vi "Read Value Defaults.vi"(11 "Effect Interface in":refnum<class "Effect Interface.lvclass">) -> (1 "Value2":T1, 2 "Value1":T1, 3 "Effect Interface out":refnum<class "Effect Interface.lvclass">)   [LabVIEW 2019, in "Effect Interface.lvlib" / "Effect Interface.lvclass"]
uses:
  Effect Interface.lvclass
  Effect Interface.lvclass/Effect Interface.ctl
  Packed Libraries/Audio Processing.lvlibp/Value Properties.ctl
  Packed Libraries/Audio Processing.lvlibp
  Packed Libraries/Audio Processing.lvlibp/Value Cluster.ctl
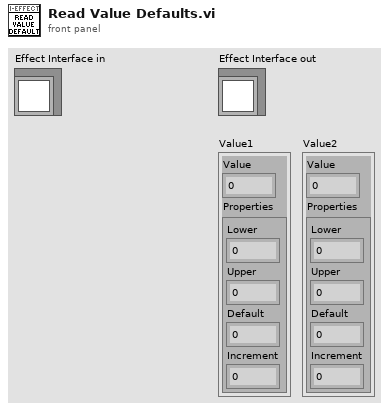
[diagram p1: front panel]
types:
  T1 = typedef "Audio Processing.lvlibp/Value Cluster.ctl" = cluster{"Value":dbl, "Properties":T2}
  T2 = typedef "Audio Processing.lvlibp/Value Properties.ctl" = cluster{"Lower":dbl, "Upper":dbl, "Default":dbl, "Increment":dbl}
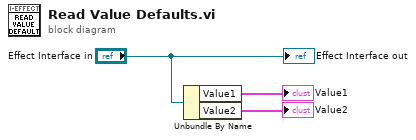
[diagram p0: block diagram]
diagram:
  n1 = Unbundle By Name("Effect Interface in") -> ("Value1"=→"Value1":T1, "Value2"=→"Value2":T1)
  "Effect Interface out" <- "Effect Interface in"
